vi "Get_Tree_Item_Data.vi"(0 "Path":path, 11 "Error In":errorcluster) -> (4 "Left Cell String":string, 6 "Child Tag":string, 15 "Error Out":errorcluster)   [LabVIEW 2026, in "Core.lvlib"]
doc: "This VI gets the data for the tree item given the path [ie tag] of the item."
uses:
  Core.lvlib
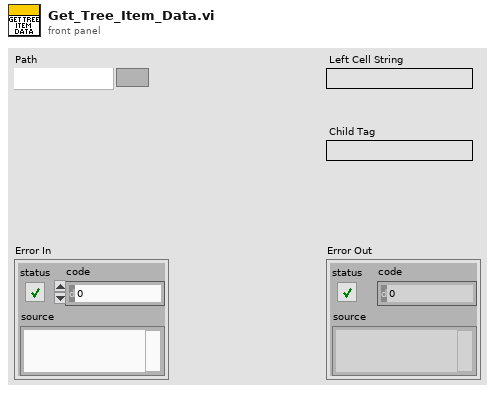
[diagram p1: front panel]
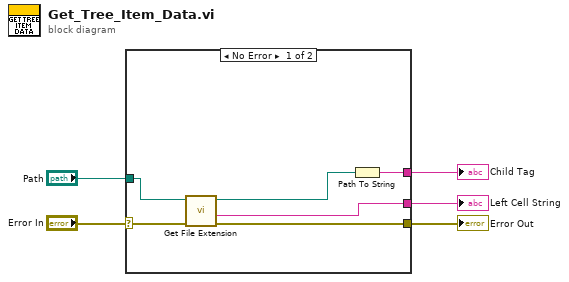
[diagram p0: block diagram]
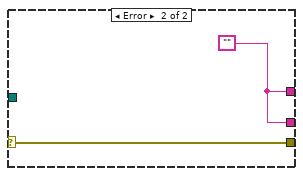
[diagram p2: hidden frame]
diagram:
  n1 = case shown="No Error" "Error In" {
    selector: "Error In" -> [w9 w13]
    tunnel: [w8 w13] -> w5
    tunnel: "Path" -> [w10 _]
    tunnel: [w7 w12] -> w3
    tunnel: [w11 w12] -> w2
    frame No Error {
      n2 = call <vilib>:"Get File Extension.vi"("error in (no error)"=w9, "file"=w10) -> ("error out"=w8:errorcluster, "filename without extension"=w7:string, "dup file"=w6:path)  [unwired: 5 in, 2 out]
      n3 = Path To String(path=w6) -> (string=w11:string)
    }
    frame Error {
      w12 = ""
    }
  }
  "Error Out" <- w5
  "Left Cell String" <- w3
  "Child Tag" <- w2
